vi "Exit With Error Cluster Code.vi"(8 "error in (no error)":errorcluster, 10 "No Error Code (0)":i32, 11 "CLI in":refnum<class "CLI.lvclass">) -> (0 "error out":errorcluster)   [LabVIEW 2015, in "CLI.lvclass"]
doc: "Exits the interface using the error cluster to determine the exit code.\n\nIf <b>error in</b> has an error this code is returned and the error message from LabVIEW.\n\nIf there is no error, exit with code 0."
uses:
  CLI.lvclass
  <vilib>/Utility/error.llb/DialogType.ctl
  Output.ctl
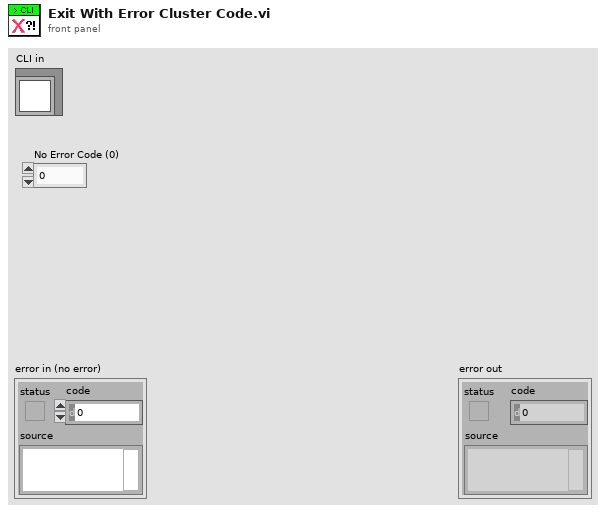
[diagram p1: front panel]
types:
  T1 = typedef "CLI.lvclass/Output.ctl" = enum16{"StdOut", "StdErr"}
  T2 = typedef "DialogType.ctl" = u16
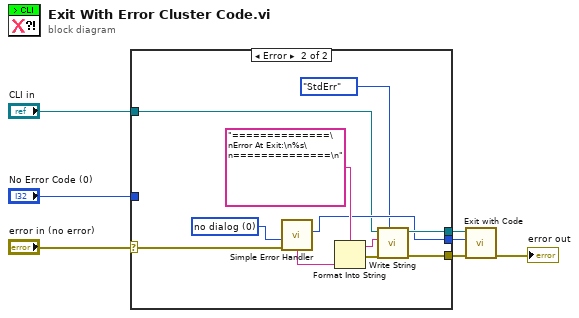
[diagram p0: block diagram]
diagram:
  n1 = case shown="Error" "error in (no error)" {
    selector: "error in (no error)" -> [w9 w12]
    tunnel: [w9 w21] -> w7
    tunnel: [w10 w20] -> w6
    tunnel: [w8 w15] -> w4
    tunnel: "CLI in" -> [w10 w13]
    tunnel: "No Error Code (0)" -> [w8 _]
    frame No Error {
    }
    frame Error {
      w19 = T2 0 items=["no dialog", "OK message", "continue or stop message", "OK message + warnings", "continue/stop + warnings"] ("type of dialog (OK msg:1)")
      n2 = call <vilib>:"Simple Error Handler.vi"("type of dialog (OK msg:1)"=w19, "error in (no error)"=w12) -> ("code out"=w15:i32, "message"=w16:string)  [unwired: 3 in, 3 out]
      n3 = Format Into String(format string="==============\nError At Exit:\n%s\n==============\n", w16) -> (resulting string=w14:string, error out=w18:errorcluster)  [unwired: 2 in]
      n4 = call "Write String.vi"("Output (StdOut)"=Output."StdErr", "error in (no error)"=w18, "Text to Write"=w14, "CLI in"=w13) -> ("error out"=w21:errorcluster, "CLI out"=w20:refnum<class "CLI.lvclass">)  [unwired: 6 in]
    }
  }
  n5 = call "Exit with Code.vi"("error in (no error)"=w7, "Exit Code (0)"=w4, "CLI in"=w6) -> ("error out"=→"error out":errorcluster)  [unwired: 8 in]
